vi "Parse Arguments.vi"(7 "Label Marker (-)":string="-", 8 "error in (no error)":errorcluster, 10 "Arguments":string[](array[string]), 11 "Option Set in":refnum<class "Option Set.lvclass">) -> (0 "error out":errorcluster, 1 "Missing Options":bool, 3 "Option Set out":refnum<class "Option Set.lvclass">, 4 "Missing Option Keys":string[](array[string]))   [LabVIEW 2015, in "Option Parser.lvlib" / "Option Set.lvclass"]
doc: "Parses the incoming arguments. After this VI you can get values for options and trailing arguments (arguments not attached to an option).\n\n<b>Label Marker</b> defines the string that comes in front of an option label. e.g. if the Label Marker is - and the label is option we will look for -option as an argument."
uses:
  Option Set.lvclass
  Option Set.lvclass/Option Set.ctl
  Option Class/Option.lvclass/Option.ctl
  <vilib>/regexp/Match Regular Expression.xnode
  Option Class/Option.lvclass
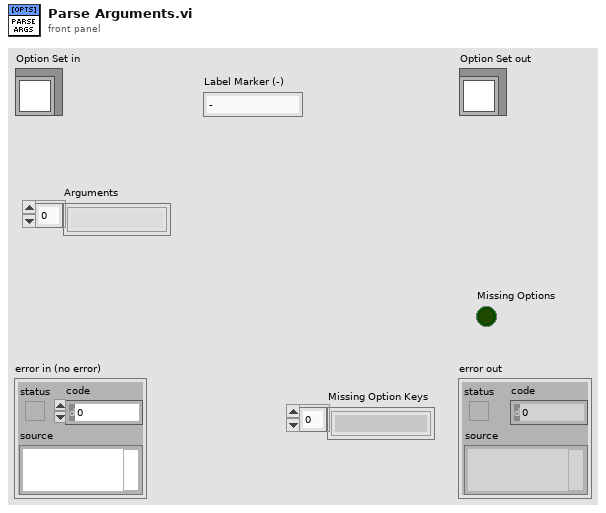
[diagram p1: front panel]
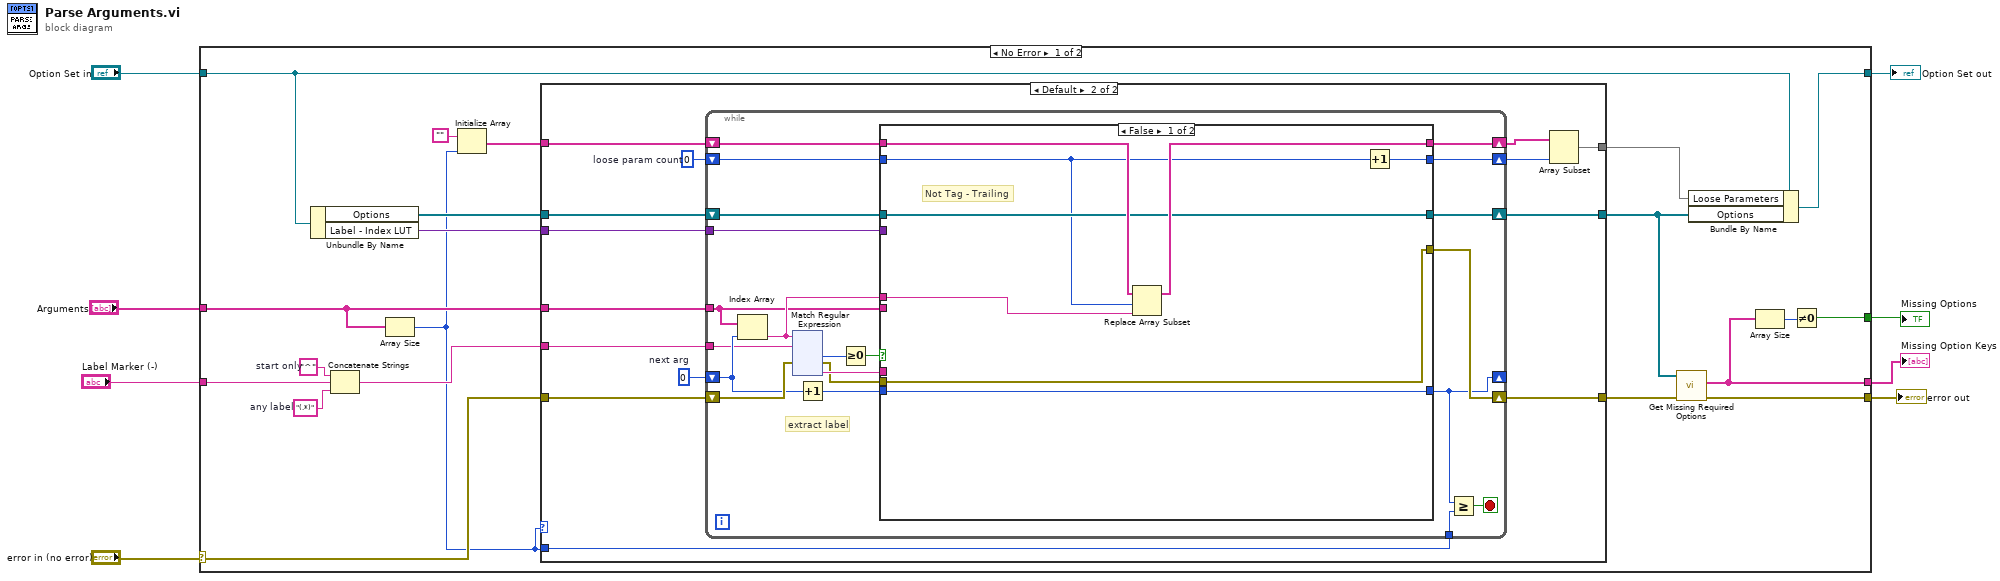
[diagram p0: block diagram]
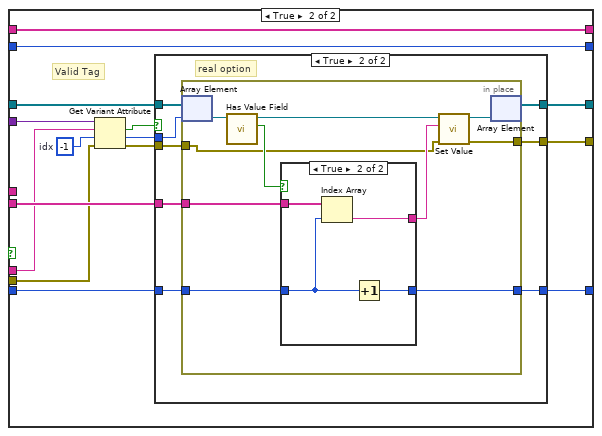
[diagram p3: hidden frame]
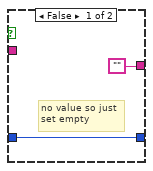
[diagram p5: hidden frame]
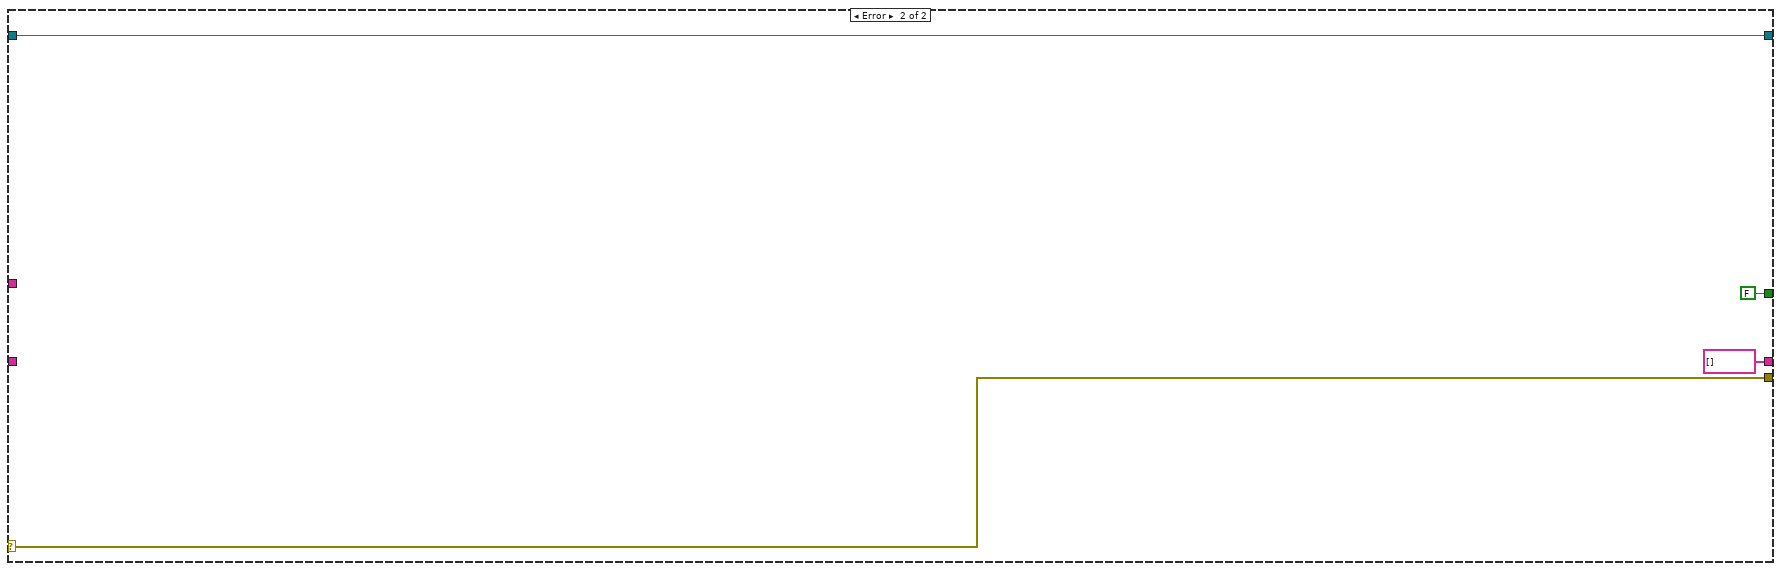
[diagram p6: hidden frame]
diagram:
  n1 = case shown="No Error" "error in (no error)" {
    selector: "error in (no error)" -> [w28 w233]
    tunnel: [w15 w233] -> w7
    tunnel: [w25 w232] -> w5
    tunnel: "Option Set in" -> [w24 w232]
    tunnel: "Arguments" -> [w23 _]
    tunnel: "Label Marker (-)" -> [w18 _]
    tunnel: [w13 string[] [] ("Missing Keys")] -> w2
    tunnel: [w11 FALSE] -> w1
    frame No Error {
      w9 = "^"  # start only
      w17 = "(.*)"  # any label
      n2 = Unbundle By Name(w24) -> ("Options"=w27:refnum<class "Option.lvclass">[], "Label - Index LUT"=w26:variant)
      n3 = Concatenate Strings(w9, w18, w17) -> (w16:string)
      n4 = Array Size(array=w23) -> (size(s)=w10:i32)
      n5 = Initialize Array("", w10) -> (w22:string[])
      n6 = case shown="Default" w10 {
        tunnel: w28 -> [w31 w44]
        tunnel: w27 -> [w30 w43]
        tunnel: w26 -> [_ w42]
        tunnel: w23 -> [_ w41]
        tunnel: w22 -> [w29 w40]
        tunnel: w10 -> [_ w39]
        tunnel: [w29 w36] -> w20
        tunnel: [w31 w34] -> w19
        tunnel: w16 -> [_ w33]
        tunnel: [w30 w32] -> w14
        frame 0 {
          # "No arguements - dont execute"
        }
        frame Default {
          w37 = 0  # loose param count
          w45 = 0  # next arg
          n7 = while {
            tunnel: w41 -> [w60]
            shift-right: [w50] -> _
            shift-left: w45 -> [w63]
            shift-right: [w59] -> w38
            shift-left: w40 -> [w58]
            shift-right: [w53] -> w32
            shift-left: w43 -> [w54]
            tunnel: w42 -> [w57]
            shift-right: [w52] -> w34
            shift-left: w44 -> [w66]
            tunnel: w39 -> [w49]
            shift-right: [w48] -> w35
            shift-left: w37 -> [w47]
            tunnel: w33 -> [w46]
            stop <- w51 stop-if-true
            # "extract label"
            n8 = Index Array(array=w60, index=w63) -> (element=w61:string)
            n9 = xnode "Match Regular Expression"("input string"=w61, "regular expression"=w46, "error in"=w66) -> ("offset past match"=w65:i32, "error out"=w55:errorcluster, "submatch 1"=w56:string)  [unwired: 3 in, 3 out]
            n10 = Increment(x=w63) -> (x+1=w62:i32)
            n11 = Greater Or Equal To 0?(x=w65) -> (x >= 0?=w64:bool)
            n12 = case shown="False" w64 {
              tunnel: w62 -> [w74 w87]
              tunnel: [w74 w86] -> w50
              tunnel: w61 -> [w69 _]
              tunnel: w60 -> [_ w88]
              tunnel: [w73 w89] -> w59
              tunnel: w58 -> [w72 w89]
              tunnel: w57 -> [_ w85]
              tunnel: w56 -> [_ w84]
              tunnel: w55 -> [w70 w82]
              tunnel: w54 -> [w71 w81]
              tunnel: [w71 w80] -> w53
              tunnel: [w70 w77] -> w52
              tunnel: [w67 w75] -> w48
              tunnel: w47 -> [w68 w75]
              frame False {
                # "Not Tag - Trailing"
                n13 = Replace Array Subset(array=w72, new element=w69, index=w68) -> (w73:string[])
                n14 = Increment(x=w68) -> (x+1=w67:i32)
              }
              frame True {
                w83 = -1  # idx
                # "Valid Tag"
                n15 = Get Variant Attribute(Variant=w85, name=w84, default value (empty Variant)=w83, error in=w82) -> (found=w76:bool, value=w79:i32, error out=w78:errorcluster)  [unwired: 1 out]
                n16 = case shown="True" w76 {
                  tunnel: w88 -> [_ w100]
                  tunnel: w87 -> [w92 w99]
                  tunnel: [w92 w98] -> w86
                  tunnel: w81 -> [w90 w97]
                  tunnel: [w90 w96] -> w80
                  tunnel: w79 -> [_ w95]
                  tunnel: w78 -> [w91 w94]
                  tunnel: [w91 w93] -> w77
                  frame False {
                  }
                  frame True {
                    # "real option"
                    n17 = in-place {
                      in-place-border: w100 -> [w110]
                      in-place-border: w99 -> [w109]
                      in-place-border: [w108] -> w98
                      in-place-border: w94 -> [w101]
                      in-place-border: [w104] -> w93
                      n18 = in-place-array #1(w97, w95) -> (w107:refnum<class "Option.lvclass">)
                      n19 = call "Has Value Field.vi"("Option in"=w107) -> ("Has Value Field"=w103:bool, "Option out"=w105:refnum<class "Option.lvclass">)  [unwired: 9 in]
                      n20 = case shown="True" w103 {
                        tunnel: w110 -> [_ w116]
                        tunnel: w109 -> [w112 w115]
                        tunnel: [w112 w114] -> w108
                        tunnel: ["" w113] -> w102
                        frame False {
                          # "no value so just\nset empty"
                        }
                        frame True {
                          n21 = Index Array(array=w116, index=w115) -> (element=w113:string)
                          n22 = Increment(x=w115) -> (x+1=w114:i32)
                        }
                      }
                      n23 = call "Set Value.vi"("error in (no error)"=w101, "Value"=w102, "Option in"=w105) -> ("error out"=w104:errorcluster, "Option out"=w106:refnum<class "Option.lvclass">)  [unwired: 7 in]
                      n24 = in-place-array #1(w106) -> (w96:refnum<class "Option.lvclass">[])  [unwired: 1 out]
                    }
                  }
                }
              }
            }
            n25 = Greater Or Equal?(x=w50, y=w49) -> (x >= y?=w51:bool)
          }
          n26 = Array Subset(array=w38, length=w35) -> (w36:string[])  [unwired: 1 in]
        }
      }
      n27 = call "Get Missing Required Options.vi"("error in (no error)"=w19, "Options"=w14) -> ("error out"=w15:errorcluster, "Missing Keys"=w13:string[])  [unwired: 8 in]
      n28 = Bundle By Name(cluster=w24, "Loose Parameters"=w20, "Options"=w14) -> (w25:refnum<class "Option Set.lvclass">)
      n29 = Array Size(array=w13) -> (size(s)=w12:i32)
      n30 = Not Equal To 0?(x=w12) -> (x != 0?=w11:bool)
    }
    frame Error {
    }
  }
  "error out" <- w7
  "Option Set out" <- w5
  "Missing Option Keys" <- w2
  "Missing Options" <- w1
